vi "set_smith_cursor_plot.vi"(6 "path":path, 7 "smith_plot":refnum<vi>, 8 "cursor_pos":i32, 9 "cursor_index":i32, 11 "plot_rjx":cluster{"array type (2D Dbl)":dbl[], dbl[]}[](array[cluster])) -> ()   [LabVIEW 2025]
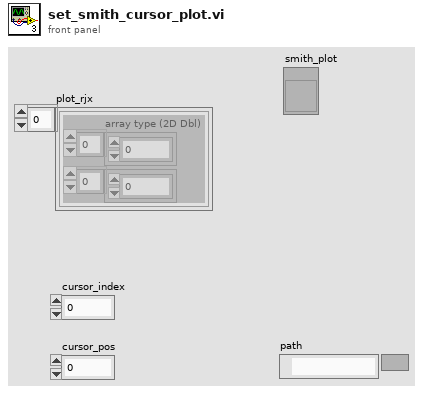
[diagram p1: front panel]
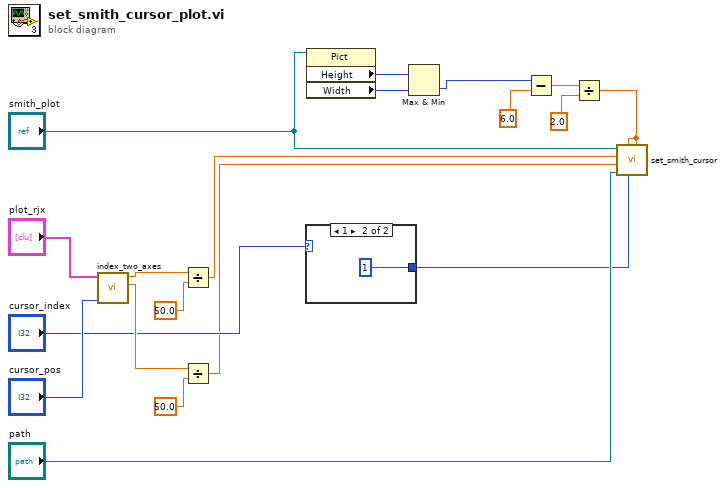
[diagram p0: block diagram]
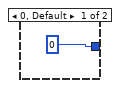
[diagram p2: hidden frame]
diagram:
  n1 = call "index_two_axes.vi"("x_index"="cursor_pos", "graph_data"="plot_rjx") -> ("Y2"=w19:dbl, "Y1"=w18:dbl)  [unwired: 7 in, 1 out]
  n2 = Divide(x=w18, y=50.0) -> (x/y=w13:dbl)
  n3 = Divide(x=w19, y=50.0) -> (x/y=w9:dbl)
  n4 = case shown="1" "cursor_index" {
    tunnel: [0 ("deco_id") 1 ("deco_id")] -> w10
    frame 0, Default {
    }
    frame 1 {
    }
  }
  n5 = property class="Pict"(reference="smith_plot") -> ("Height"=w4:u32, "Width"=w3:u32)  [unwired: 1 in, 2 out]
  n6 = Max & Min(x=w4, y=w3) -> (min(x,y)=w2:u32)  [unwired: 1 out]
  n7 = Subtract(x=w2, y=6.0) -> (x-y=w6:dbl)
  n8 = Divide(x=w6, y=2.0) -> (x/y=w1:dbl)
  n9 = call "set_smith_cursor.vi"("left_center"=w1, "deco_id"=w10, "top_center"=w1, "vi path"="path", "x"=w9, "r"=w13, "show_plot_ref"="smith_plot") -> ()  [unwired: 5 in]
